vi "Get_Last_Error.vi"(8 "error in (no error)":errorcluster, 11 "muExpr in":refnum<class "mupExpr.lvclass">) -> (0 "error out":errorcluster, 2 "error details":T1, 3 "muExpr out":refnum<class "mupExpr.lvclass">)   [LabVIEW 2018, in "mupExpr.lvclass"]
doc: "Return the details of the last error that occured"
uses:
  mupExpr.lvclass
  mupExpr.lvclass/mupExpr.ctl
  mupLib/mupLib.lvlib
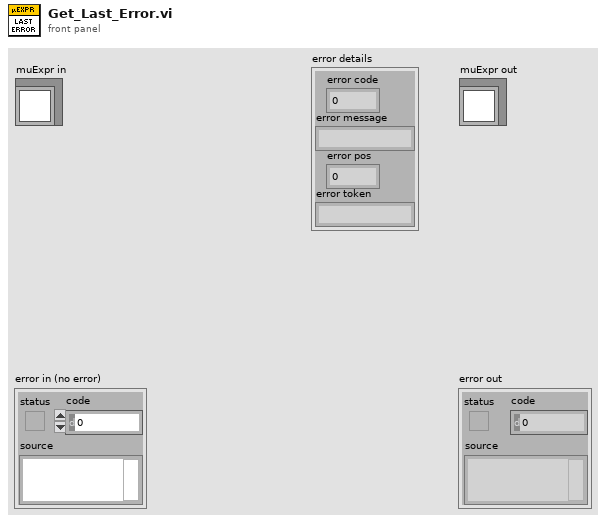
[diagram p1: front panel]
types:
  T1 = cluster{"error code":i32, "error message":string, "error pos":i32, "error token":string}
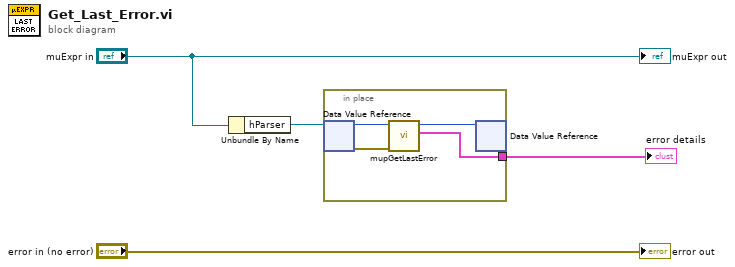
[diagram p0: block diagram]
diagram:
  n1 = Unbundle By Name("muExpr in") -> ("hParser"=w1:refnum<data-value>)
  n2 = in-place {
    in-place-border: [w8] -> w3
    n3 = in-place-dvr #1(w1) -> (w6:u64, w7:errorcluster)
    n4 = call "mupGetLastError.vi"("error in (no error)"=w7, "hParser in"=w6) -> ("error details"=w8:T1, "hParser out"=w5:u64)  [unwired: 7 in, 1 out]
    n5 = in-place-dvr #1(w5) -> ()  [unwired: 2 out]
  }
  "error details" <- w3
  "error out" <- "error in (no error)"
  "muExpr out" <- "muExpr in"
